vi "Crc calculator.vi"(9 "unsigned byte array":u8[](array[numeric]), 10 "Polynom":u16=4129 format="%.0x", 11 "ReverseCRC":bool) -> (3 "CRC Value":u16 format="%.0x")   [LabVIEW 2020]
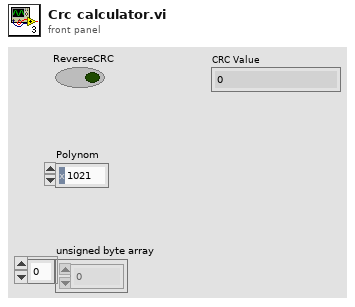
[diagram p1: front panel]
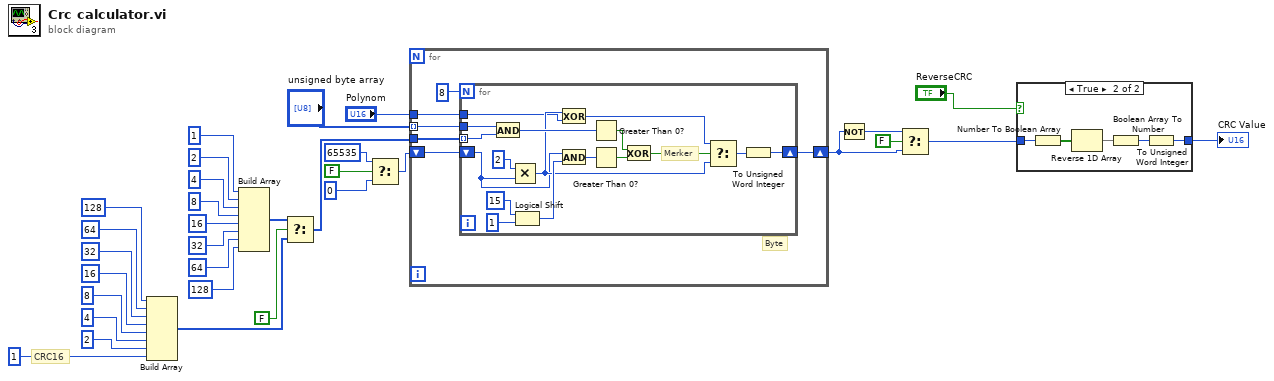
[diagram p0: block diagram]
diagram:
  # "CRC16"
  n1 = Build Array(u8 128, u8 64, u8 32, u8 16, u8 8, u8 4, u8 2, u8 1) -> (w20:u8[])
  n2 = Build Array(u8 1, u8 2, u8 4, u8 8, u8 16, u8 32, u8 64, u8 128) -> (w21:u8[])
  n3 = Select(t=w21, s=FALSE, f=w20) -> (s? t:f=w19:u8[])
  n4 = Select(t=u16 65535, s=FALSE, f=u16 0) -> (s? t:f=w2:u16)
  n5 = for {
    shift-right: [w36] -> w24
    shift-left: w2 -> [w38]
    tunnel: "unsigned byte array" -> [w35] mode=indexing
    tunnel: w19 -> [w34]
    tunnel: "Polynom" -> [w33]
    # "Byte"
    n6 = for {
      N: 8 -> [_]
      shift-right: [w54] -> w36
      shift-left: w38 -> [w44]
      tunnel: w34 -> [w45] mode=indexing
      tunnel: w35 -> [w40]
      tunnel: w33 -> [w39]
      # "Merker"
      n7 = And(x=w40, y=w45) -> (x .and. y?=w52:u8)
      n8 = Multiply(x=u16 2, y=w44) -> (x*y=w46:u16)
      n9 = Logical Shift(y=u16 15, x=u16 1) -> (x << y=w48:u16)
      n10 = Exclusive Or(1:w39, 2:w46) -> (0:w55:u16)
      n11 = And(x=w44, y=w48) -> (x .and. y?=w47:u16)
      n12 = Greater Than 0?(x=w52) -> (x > 0?=w51:bool)
      n13 = Greater Than 0?(x=w47) -> (x > 0?=w42:bool)
      n14 = Exclusive Or(1:w42, 2:w51) -> (0:w41:bool)
      n15 = Select(t=w55, s=w41, f=w46) -> (s? t:f=w53:u16)
      n16 = To Unsigned Word Integer(number=w53) -> (unsigned 16bit integer=w54:u16)
    }
  }
  n17 = Not(x=w24) -> (.not. x?=w25:u16)
  n18 = Select(t=w25, s=FALSE, f=w24) -> (s? t:f=w26:u16)
  n19 = case shown="True" "ReverseCRC" {
    tunnel: w26 -> [w56 w61]
    tunnel: [w56 w57] -> w28
    frame False {
    }
    frame True {
      n20 = Number To Boolean Array(number=w61) -> (Boolean array=w60:bool[])
      n21 = Reverse 1D Array(array=w60) -> (reversed array=w59:bool[])
      n22 = Boolean Array To Number(Boolean array=w59) -> (number=w58:u32)
      n23 = To Unsigned Word Integer(number=w58) -> (unsigned 16bit integer=w57:u16)
    }
  }
  "CRC Value" <- w28
